vi "RemoteVI Service Clients.vi"(0 "clients":T2(array[cluster]), 1 "windows":T3(array[cluster]), 5 "geo":T4, 7 "hWnd":u64, 9 "popups":T1) -> (4 "clients out":T2(array[cluster]), 6 "popups out":T1, 8 "clicked?":bool)   [LabVIEW 2020, in "RemoteVI.lvlib"]
doc: "Services every client once (RemoteVI Service Client.vi), in order: reads and handles what each one sent. popups travels from client to client, so a displacement d set by a popup click of one client applies to the next; popups out carries the last one. clicked? is TRUE when any client posted a message that may open a LabVIEW popup. No VI Server call; geo, hWnd and windows (the application's other windows, docs\\protocol.md section 7) come from the server loop's cache."
uses:
  RemoteVI.lvlib
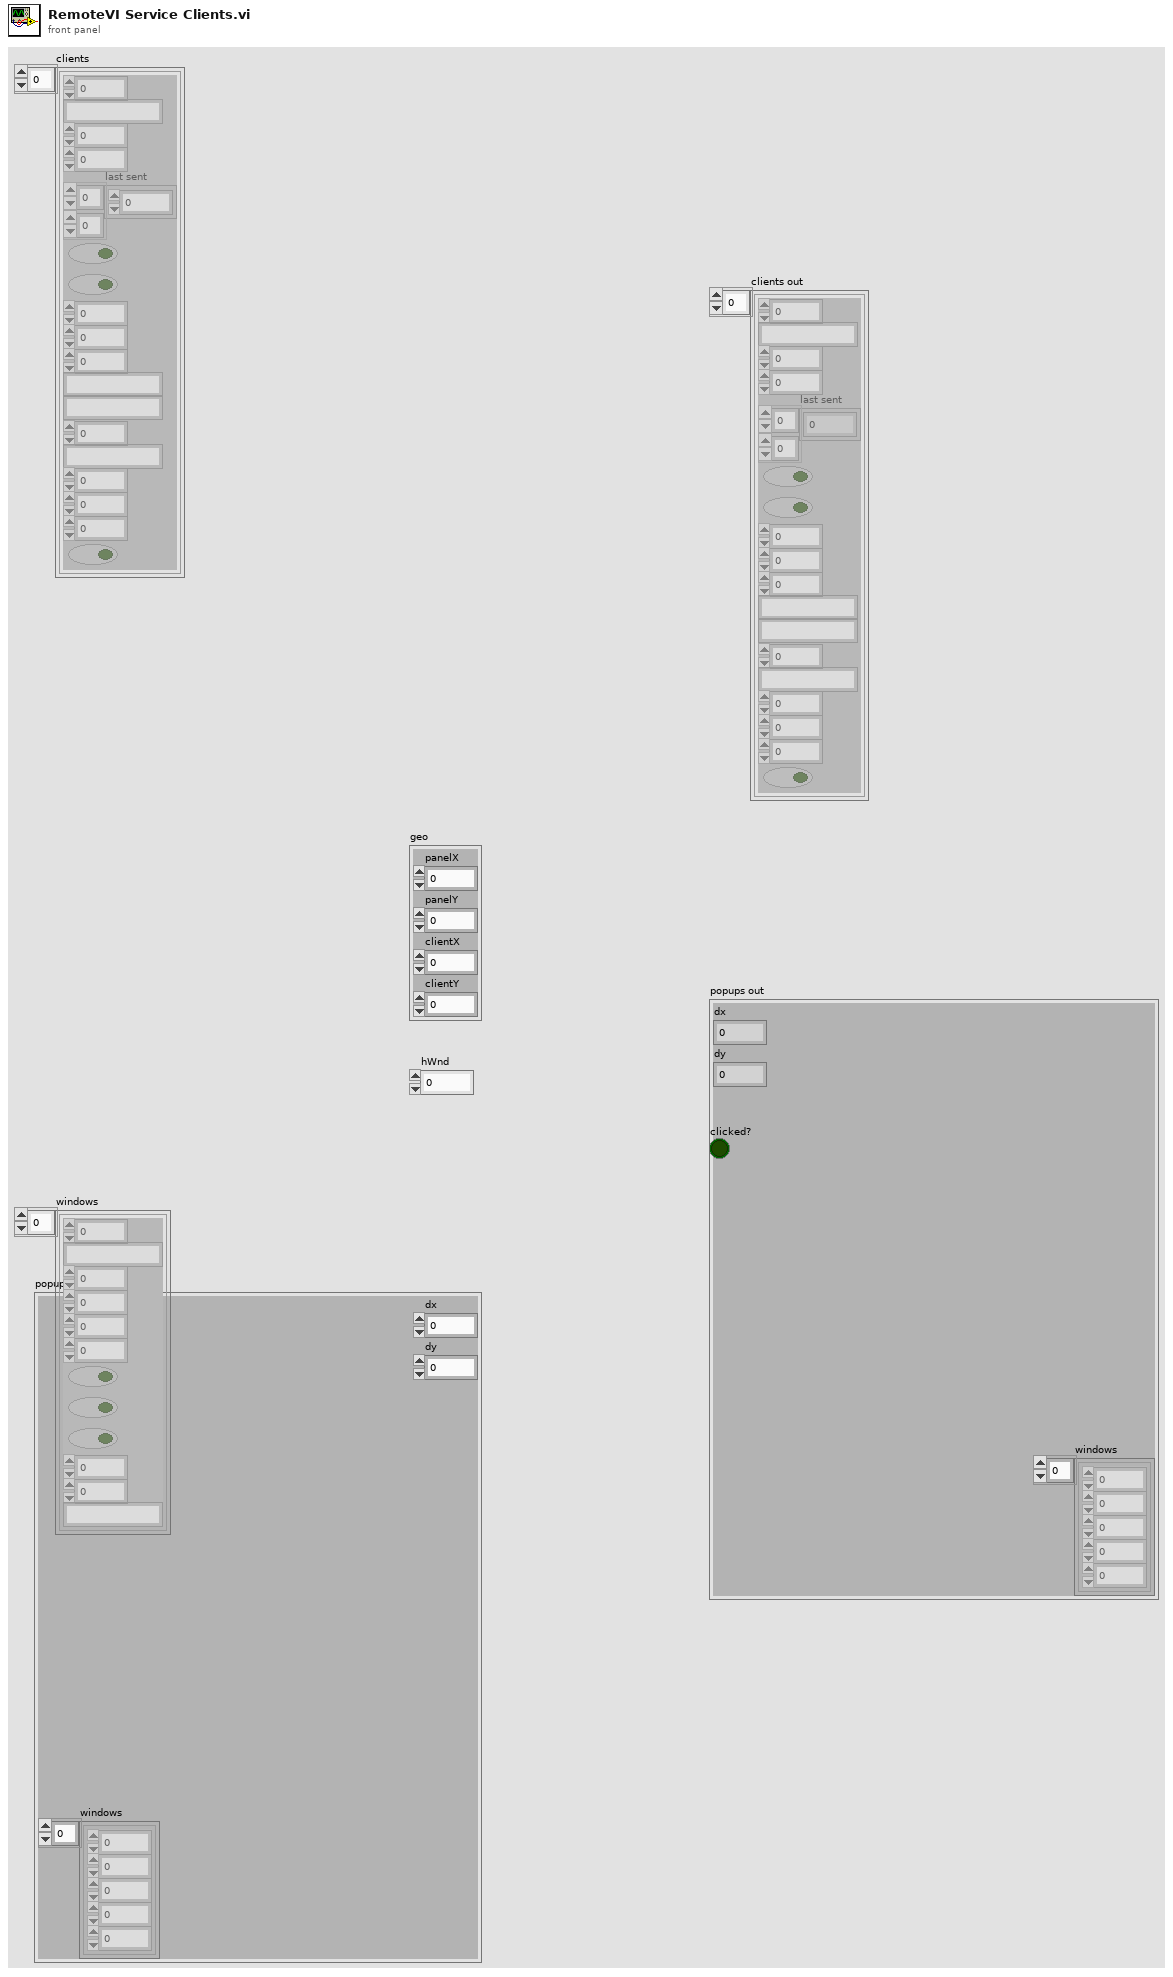
[diagram p1: front panel]
types:
  T1 = cluster{"windows":cluster{"hwnd":u64, "x":i32, "y":i32, "w":i32, "h":i32}[], "dx":i32, "dy":i32}
  T2 = cluster{"connection":u32, "rx buffer":string, "seq":u32, "acked":u32, "last sent":u32[][], "tracking":bool, "closed":bool, "mods":u8, "mods set":u8, "popup since":u32, "windows sent":string, "window frames":cluster{"id":u64, "pixels":u32[][]}[], "key window":u64, "address":string, "since":dbl, "last input":dbl, "bytes":dbl, "view only":bool}[]
  T3 = cluster{"id":u64, "title":string, "x":i32, "y":i32, "w":i32, "h":i32, "modal":bool, "active":bool, "closable":bool, "sx":i32, "sy":i32, "class":string}[]
  T4 = cluster{"panelX":i32, "panelY":i32, "clientX":i32, "clientY":i32}
  T5 = cluster{"connection":u32, "rx buffer":string, "seq":u32, "acked":u32, "last sent":u32[][], "tracking":bool, "closed":bool, "mods":u8, "mods set":u8, "popup since":u32, "windows sent":string, "window frames":cluster{"id":u64, "pixels":u32[][]}[], "key window":u64, "address":string, "since":dbl, "last input":dbl, "bytes":dbl, "view only":bool}
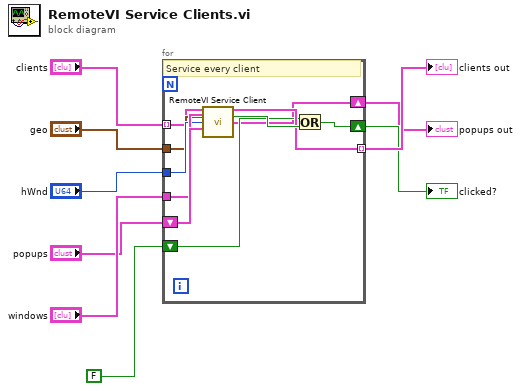
[diagram p0: block diagram]
diagram:
  n1 = for {
    tunnel: "clients" -> [w10] mode=indexing
    tunnel: "geo" -> [w11]
    tunnel: "hWnd" -> [w12]
    tunnel: "windows" -> [w13]
    shift-right: [w15] -> w7
    shift-left: "popups" -> [w14]
    shift-right: [w17] -> w8
    shift-left: FALSE -> [w16]
    tunnel: [w18] -> w9 mode=indexing
    # "Service every client"
    n2 = call "RemoteVI Service Client.vi"("Client"=w10, "windows"=w13, "geo"=w11, "hWnd"=w12, "popups"=w14) -> ("Client out"=w18:T5, "clicked?"=w19:bool, "popups out"=w15:T1)  [unwired: 7 in, 1 out]
    n3 = Or(x=w16, y=w19) -> (x .or. y?=w17:bool)
  }
  "clients out" <- w9
  "popups out" <- w7
  "clicked?" <- w8
